vi "Do.vi"(8 "error in (no error)":errorcluster, 10 "Actor in":refnum<class "Actor.lvclass">, 11 "Run Msg":refnum<class "Run Msg.lvclass">) -> (0 "error out":errorcluster, 2 "Actor out":refnum<class "Actor.lvclass">)   [LabVIEW 2026, in "IRunner.lvlib" / "Run Msg.lvclass"]
doc: "This VI delivers the message to the actor by calling the appropriate method(s) on the actor."
uses:
  Run Msg.lvclass
  Run Msg.lvclass/Run Msg.ctl
  9ef47adc-f318-494c-9b8b-6df3216d6863.vi
  IRunner/IRunner.lvclass
  <vilib>/ActorFramework/Actor/Actor.lvclass
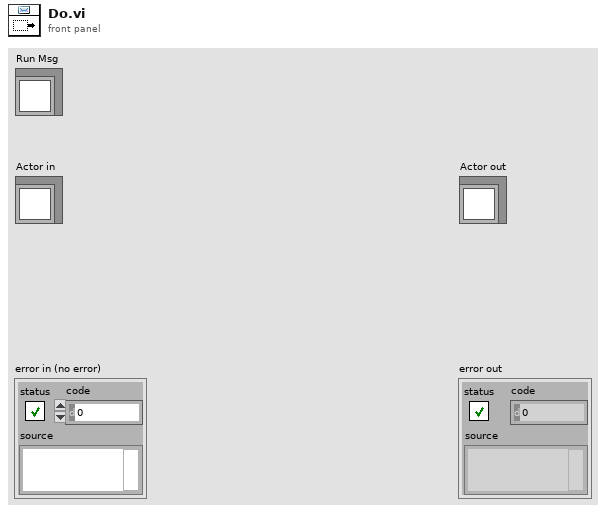
[diagram p1: front panel]
types:
  T1 = typedef "NI_App_Builder_API.lvlib/Build Specification Version.ctl" = cluster{"Major":u16, "Minor":u16, "Fix":u16, "Build":u16}
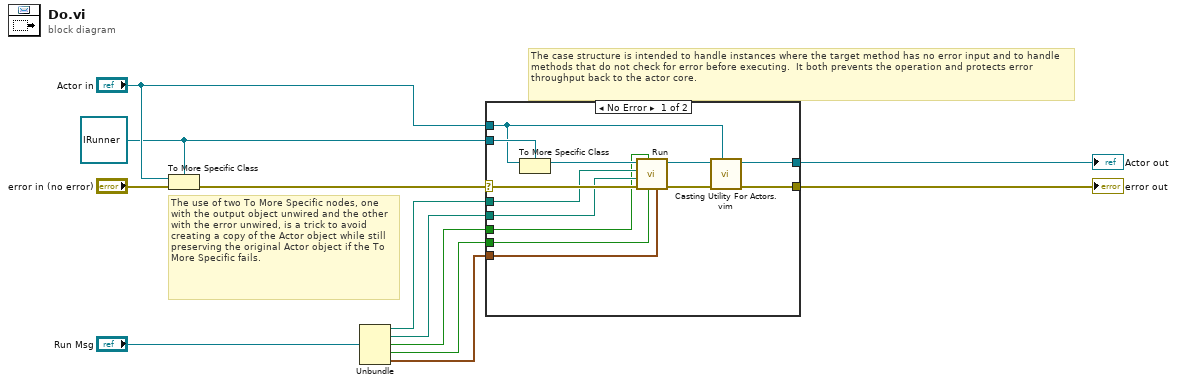
[diagram p0: block diagram]
diagram:
  w6 = refnum<class "IRunner.lvclass"> refnum ("Actor in")
  # "The use of two To More Specific nodes, one with the output object unwired and the other with the error unwired, is a trick to avoid creating a copy of the Actor object while still preserving the original Actor object if the To More Specific fails."
  # "The case structure is intended to handle instances where the target method has no error input and to handle methods that do not check for error before executing.  It both prevents the operation and protects error throughput back to the actor core."
  n1 = To More Specific Class(target class=w6, reference="Actor in", error in="error in (no error)") -> (error out=w10:errorcluster)  [unwired: 1 out]
  n2 = Unbundle("Run Msg") -> (w5:path, w4:path, w3:bool, w2:bool, w1:T1)
  n3 = case shown="No Error" w10 {
    selector: w10 -> [w25 w27]
    tunnel: [w19 w27] -> w9
    tunnel: [w20 w26] -> w8
    tunnel: "Actor in" -> [w22 w26]
    tunnel: w6 -> [w23 _]
    tunnel: w5 -> [w17 _]
    tunnel: w4 -> [w16 _]
    tunnel: w3 -> [w15 _]
    tunnel: w2 -> [w14 _]
    tunnel: w1 -> [w13 _]
    frame No Error {
      n4 = To More Specific Class(target class=w23, reference=w22) -> (specific class reference=w24:refnum<class "IRunner.lvclass">)  [unwired: 1 in, 1 out]
      n5 = call-dynamic "Run.vi"("Build Specification Version"=w13, "Set PPL Version"=w14, "Clear Compiled Object Cache"=w15, "error in"=w25, "Python Module"=w16, "Output Folder"=w17, "IRunner in"=w24) -> ("error out"=w18:errorcluster, "IRunner out"=w21:refnum<class "IRunner.lvclass">)  [unwired: 3 in]
      n6 = call "Casting Utility For Actors.vim"("type"=w22, "error in (no error)"=w18, "Actor in"=w21) -> ("error out"=w19:errorcluster, "Actor out"=w20:refnum<class "Actor.lvclass">)  [unwired: 7 in]
    }
    frame Error {
      # "If type check fails, pass the original object out again."
    }
  }
  "error out" <- w9
  "Actor out" <- w8
